vi "CSM-INI Variable Viewer - DebugTool.vi"(7 "Current Module(\"\" to generate an ID)":string="IniViewer") -> ()   [LabVIEW 2017]
doc: "CSM INI-Variable is a global configuration information. This tool is used to view and debug the current configuration information in memory.\n\n\n> [!NOTE] <b>CSM INI-Variable Addon</b>\n>\n> Configuration files are an essential component of application development. The CSM INI-Variable Addon provides simple and easy-to-use configuration file support for CSM, allowing users to configure applications without explicitly reading or writing configuration files.\n>\n> CSM INI-Variable configuration file data uses the CSM API String format.\n>\n> The following are key features:\n> 1. <b>Default Configuration Handling</b>: Automatically loads the default configuration file upon the first library function call, eliminating the need for explicit user loading.\n> 2. <b>Multi-File Support</b>: Supports loading multiple configuration files via specialized functions.\n> 3. <b>Memory Caching</b>: Maintains a cached copy in memory. Applications retrieve configuration information from this cache.\n> 4. <b>INI Format Compatibility</b>: Both configuration files and the memory copy use the standard INI format, supporting sections and key-value pairs.\n> 5. <b>Efficient Caching Mechanism</b>: Optimizes performance using a global modification flag, re-reading the memory copy only when the configuration has been modified.\n>\n> This library includes and utilizes a copy of [LabVIEW-Config](https://github.com/rcpacini/LabVIEW-Config) developed by [@rcpacini](https://github.com/rcpacini)."
uses:
  <userlib>/_NEVSTOP/Communicable State Machine(CSM)/_tool/_csmlite/_PassAllowedMessage - MsgList.vi
  _csm-iniViewer/csm-iniViewer.lvlib
  INI-Static-Variable-Support/INI-Static-Variable-Support.lvlib
  <userlib>/_NEVSTOP/Communicable State Machine(CSM)/_tool/_csmlite/_csmlite.lvlib
  <userlib>/_NEVSTOP/Communicable State Machine(CSM)/_tool/_ui/csm-ui-support.lvlib
panel:
  in  "Close":bool
  in  "Remove all Configurations":bool
  in  "Open":bool
  in  "Refresh":bool
  in  "Include Value?":bool
  in  "Filter":string
  in  "Tree":string(tree)
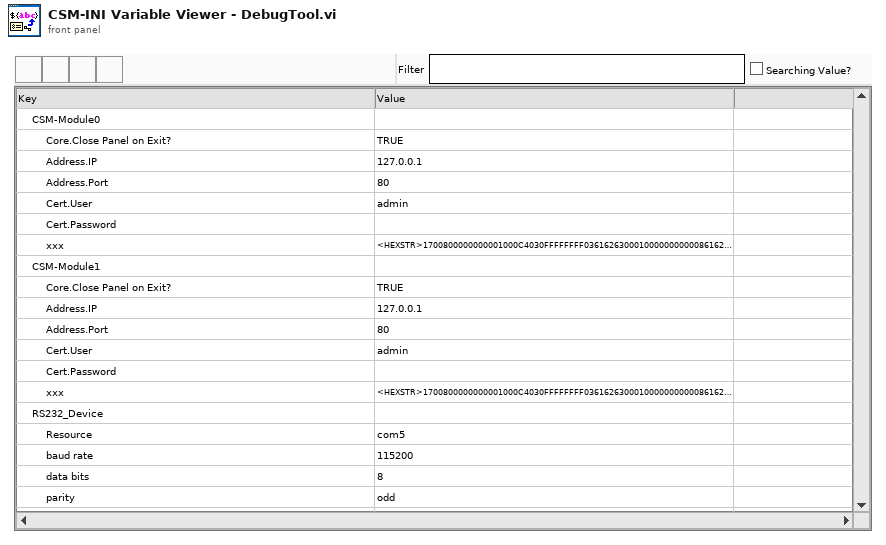
[diagram p1: front panel]
types:
  T1 = enum32{"Invalid", "Standard", "Closed", "Hidden", "Minimized", "Maximized"}
  T2 = enum32{"invalid app kind", "Development System", "Run Time System", "Student Edition", "Embedded LabVIEW", "Evaluation", "Custom"}
  T3 = cluster{"Core":cluster{"Current VI Reference":refnum<vi>, "Close Panel on Exit?":bool}, "Your Boolean data":bool, "Your string data":string}
  T4 = cluster{"Current VI Reference":refnum<vi>, "Close Panel on Exit?":bool}
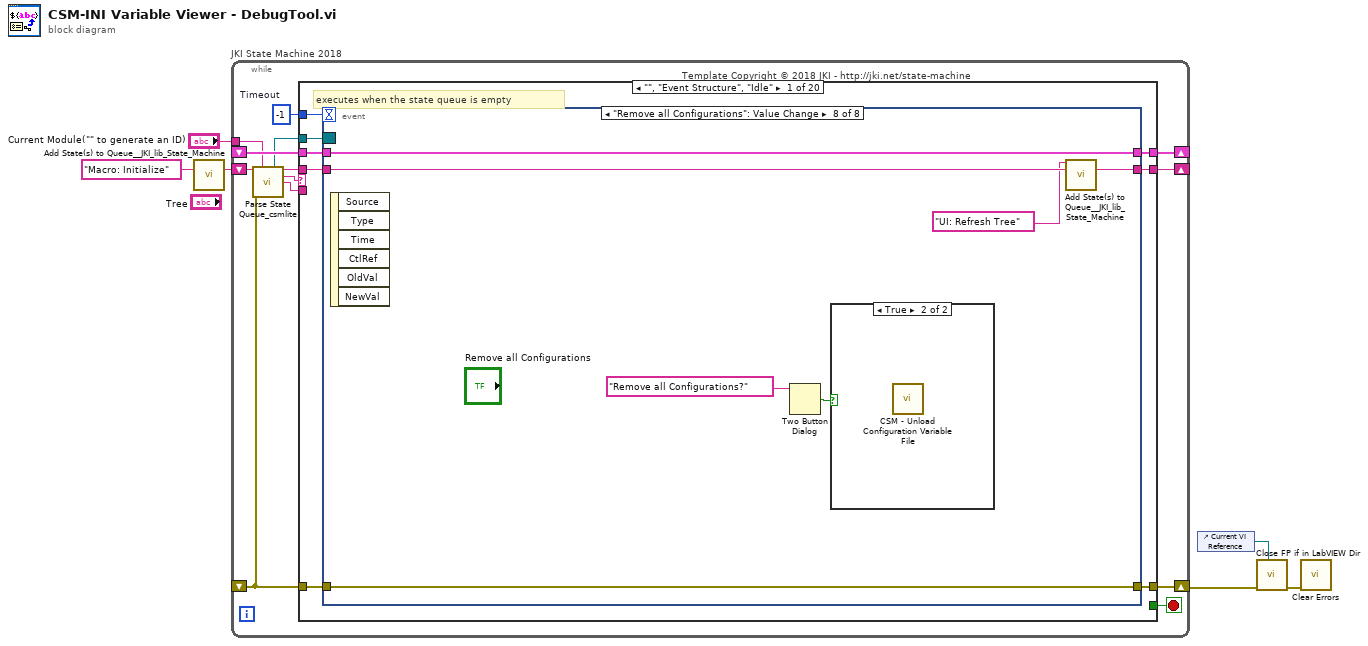
[diagram p0: block diagram]
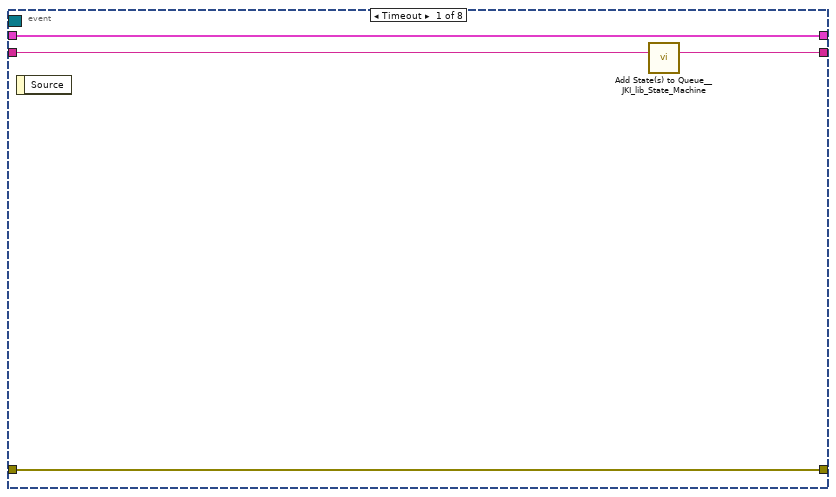
[diagram p2: hidden frame]
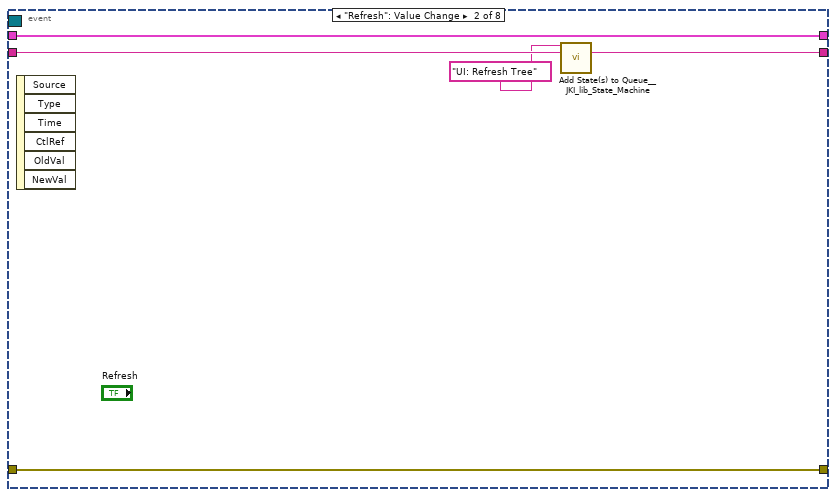
[diagram p3: hidden frame]
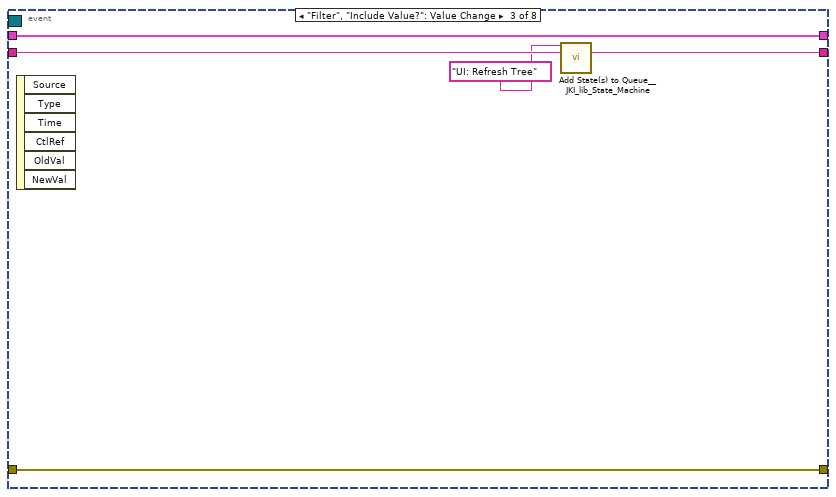
[diagram p4: hidden frame]
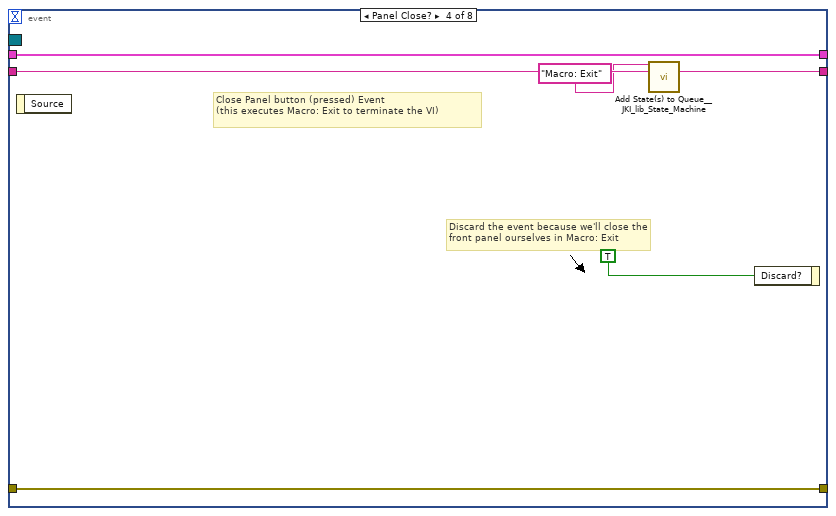
[diagram p5: hidden frame]
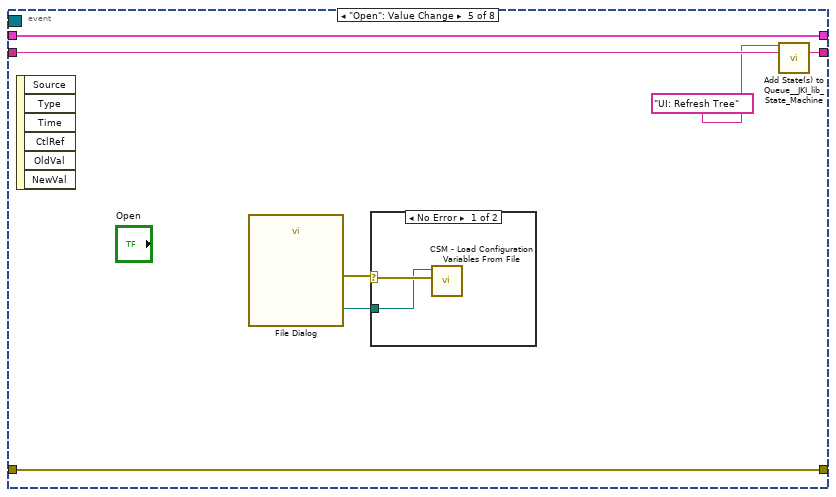
[diagram p6: hidden frame]
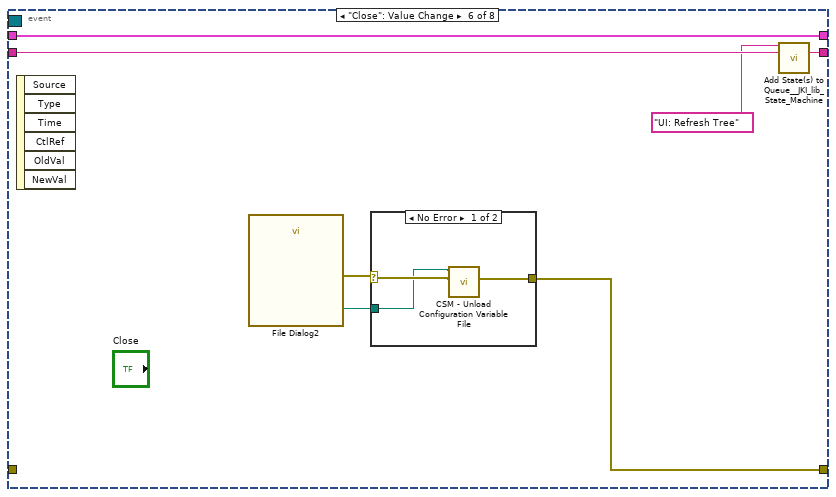
[diagram p8: hidden frame]
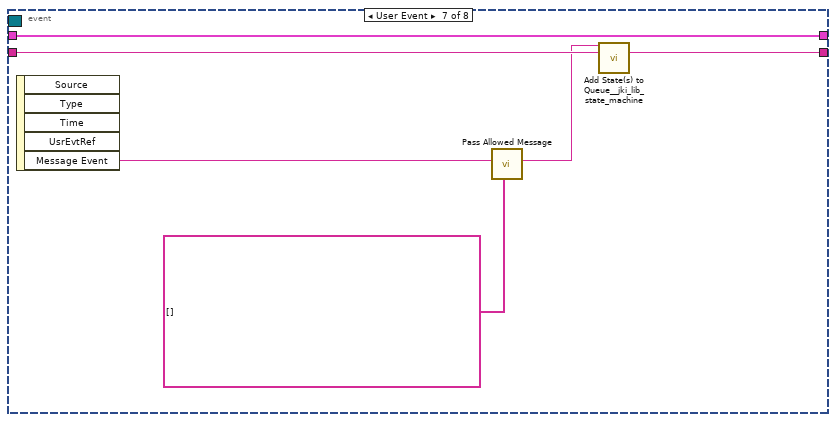
[diagram p10: hidden frame]
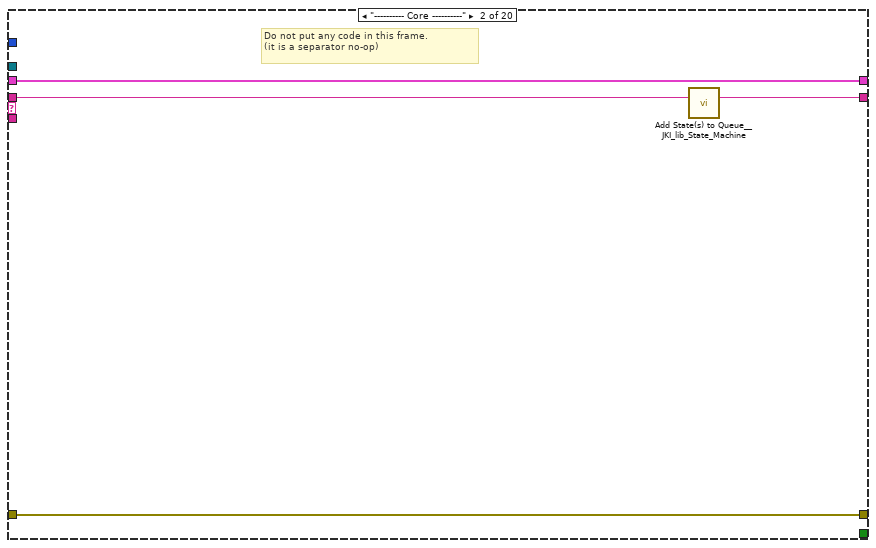
[diagram p12: hidden frame]
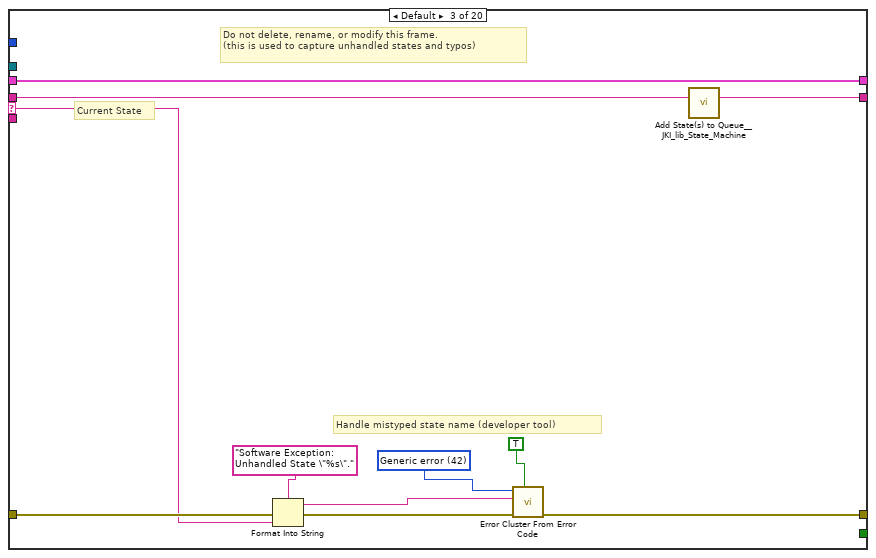
[diagram p13: hidden frame]
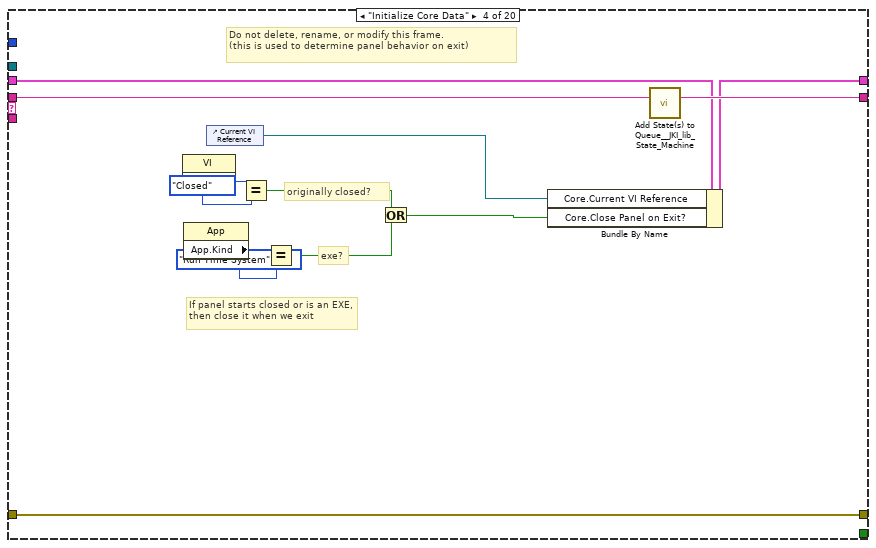
[diagram p14: hidden frame]
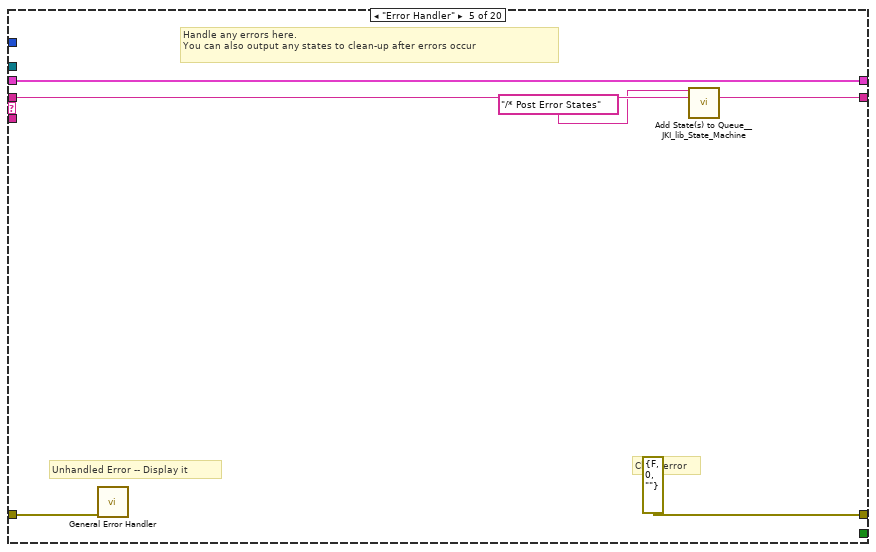
[diagram p15: hidden frame]
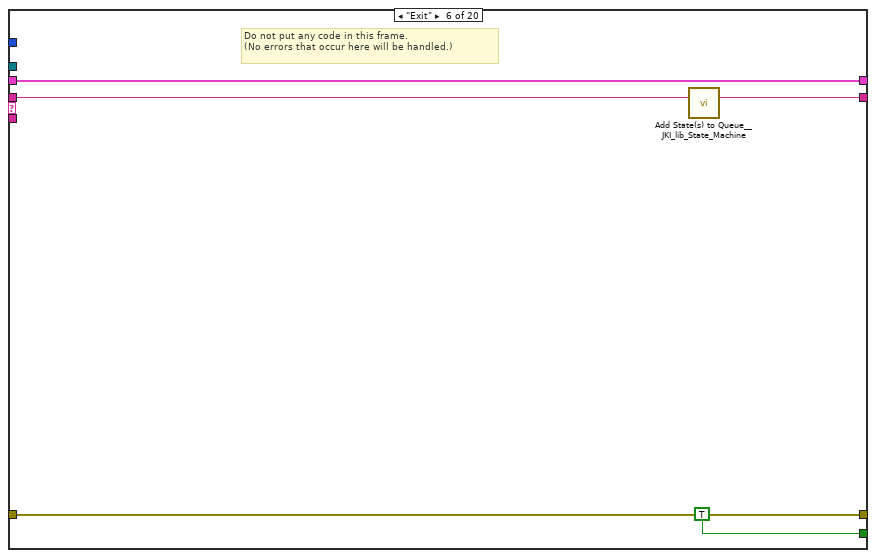
[diagram p16: hidden frame]
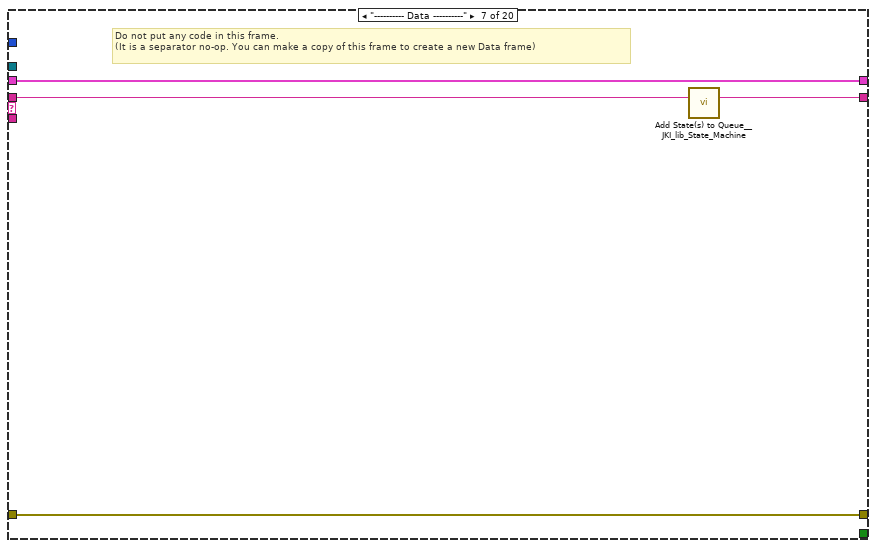
[diagram p17: hidden frame]
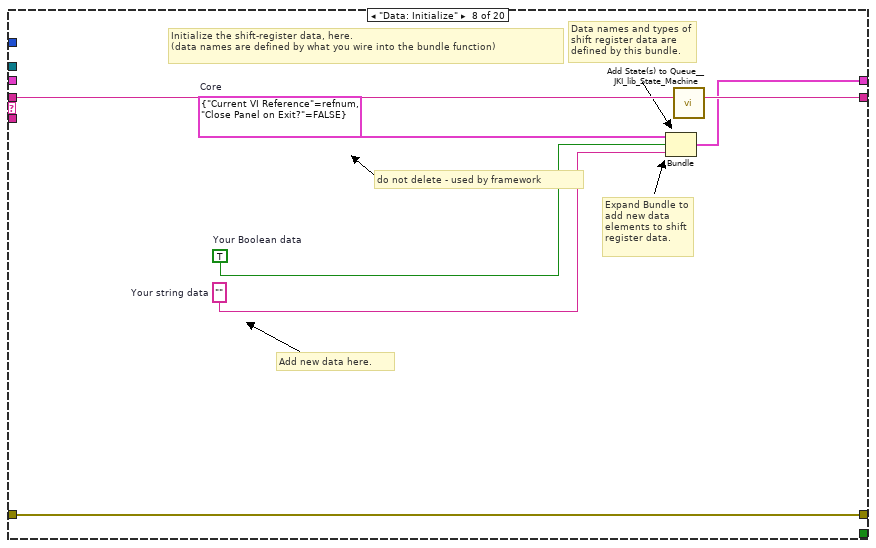
[diagram p18: hidden frame]
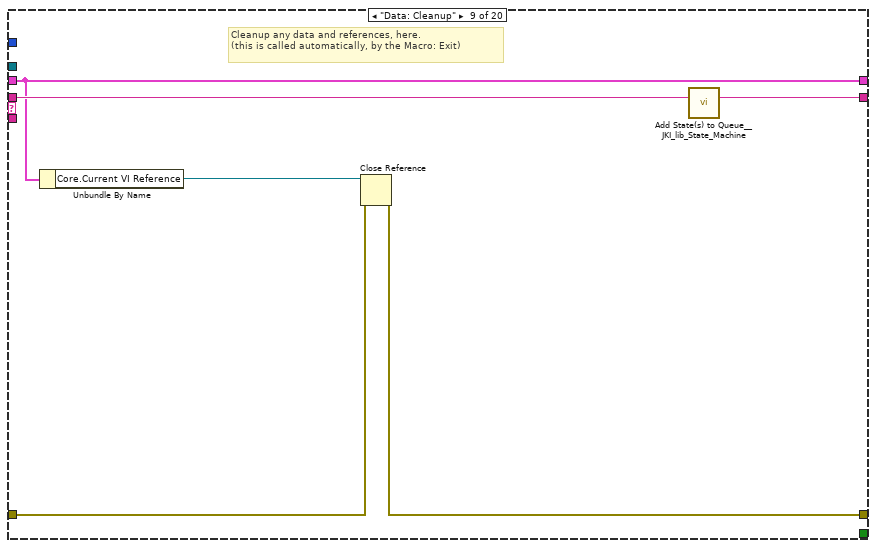
[diagram p19: hidden frame]
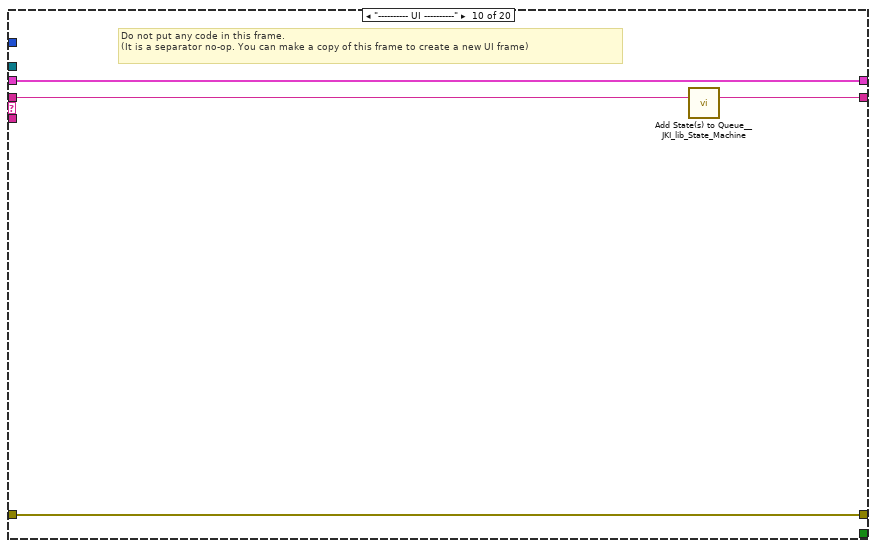
[diagram p20: hidden frame]
diagram:
  n1 = call <vilib>:"Add State(s) to Queue__JKI_lib_State_Machine.vi"("State(s) in (\"\")"="Macro: Initialize") -> ("States Out"=w6:string)  [unwired: 14 in]
  n2 = while "JKI State Machine 2018" {
    shift-right: [w12] -> _
    shift-left: _ -> [w11]
    shift-right: [w15] -> w3
    shift-left: _ -> [w9]
    shift-right: [w14] -> _
    shift-left: w6 -> [w16]
    tunnel: "Current Module(\"\" to generate an ID)" -> [w8]
    stop <- w13 stop-if-true
    w10 = -1  # Timeout
    # "Template Copyright © 2018 JKI - http://jki.net/state-machine"
    n3 = call <userlib>:"Parse State Queue_csmlite.vi"("State Queue"=w16, "Current Module(\"\" to generate an ID)"=w8, "Error In (no error)"=w9) -> ("Event Registration Refnum"=w7:refnum<event-registration>, "Remaining States"=w18:string, "Current State"=w19:string, "Arguments"=w17:string)  [unwired: 9 in]
    n4 = case shown="\"\", \"Event Structure\", \"Idle\"" w19 {
      selector: w19 -> [_ _ w84 _ _ _ _ _ _ _ _ _ _ _ _ _ _ _ _ _]
      tunnel: w18 -> [w27 w83 w88 w107 w113 w118 w122 w129 w135 w139 w151 w157 w168 w239 w243 w248 w258 w262 w266 w270]
      tunnel: w17 -> [_ _ _ _ _ _ _ _ _ _ _ w152 w162 _ _ _ _ _ _ _]
      tunnel: w11 -> [w25 w80 w86 w100 w110 w116 w119 _ w130 w136 w149 w155 w164 w238 w240 w245 w255 w259 w263 w267]
      tunnel: [w24 w81 w90 w104 errorcluster {"status"=FALSE, "code"=0, "source"=""} ("error out") w115 w120 w126 w131 w137 w148 w153 w165 w235 w241 w246 w256 w260 w264 w268] -> w15
      tunnel: w9 -> [w23 w81 w89 w104 w109 w115 w120 w126 w132 w137 w148 w154 w166 _ w241 w246 w256 w260 w264 w268]
      tunnel: [w26 w82 w87 w106 w112 w117 w121 w128 w134 w138 w150 w156 w167 w239 w242 w247 w257 w261 w265 w269] -> w14
      tunnel: [_ _ _ _ _ TRUE _ _ _ _ _ _ _ _ _ _ _ _ _ _] -> w13
      tunnel: [w22 w80 w86 w105 w110 w116 w119 w127 w130 w136 w149 w155 w164 w238 w240 w245 w255 w259 w263 w267] -> w12
      tunnel: w10 -> [w21 _ _ _ _ _ _ _ _ _ _ _ _ _ _ _ _ _ _ _]
      tunnel: w7 -> [w20 _ _ _ _ _ _ _ _ _ _ _ _ _ _ _ _ _ _ _]
      frame "", "Event Structure", "Idle" {
        # "executes when the state queue is empty"
        n5 = event shown="[7] \"Remove all Configurations\": Value Change" {
          selector: w20 -> [_ _ _ _ _ _ _ _]
          dyn-events: _ -> [_ _ _ _ _ _ _ _]
          timeout: w21 -> [_ _ _ _ _ _ _ _]
          tunnel: w27 -> [w31 w34 w39 w47 w49 w59 w68 w76]
          tunnel: [w30 w35 w40 w46 w50 w60 w69 w77] -> w26
          tunnel: w25 -> [w28 w36 w41 w44 w54 w63 w72 w79]
          tunnel: [w29 w32 w37 w45 w53 w57 _ w78] -> w24
          tunnel: w23 -> [w29 w32 w37 w45 w53 _ _ w78]
          tunnel: [w28 w36 w41 w44 w54 w63 w72 w79] -> w22
          event Timeout {
            n6 = event-data() -> ()  [unwired: 1 in, 1 out]
            n7 = call <vilib>:"Add State(s) to Queue__JKI_lib_State_Machine.vi"("State(s) in (\"\")"=w31) -> ("States Out"=w30:string)  [unwired: 14 in]
          }
          event "Refresh": Value Change {
            n8 = event-data() -> ()  [unwired: 1 in, 6 out]
            n9 = call <vilib>:"Add State(s) to Queue__JKI_lib_State_Machine.vi"("State(s) in Front (\"\")"="UI: Refresh Tree" ("State(s) in Front (\"\")"), "State(s) in (\"\")"=w34) -> ("States Out"=w35:string)  [unwired: 13 in]
          }
          event "Filter", "Include Value?": Value Change {
            n10 = event-data() -> ()  [unwired: 1 in, 6 out]
            n11 = call <vilib>:"Add State(s) to Queue__JKI_lib_State_Machine.vi"("State(s) in Front (\"\")"="UI: Refresh Tree" ("State(s) in Front (\"\")"), "State(s) in (\"\")"=w39) -> ("States Out"=w40:string)  [unwired: 13 in]
          }
          event Panel Close? {
            # "Discard the event because we'll close the front panel ourselves in Macro: Exit"
            # "Close Panel button (pressed) Event\n(this executes Macro: Exit to terminate the VI)"
            n12 = event-data() -> ()  [unwired: 1 in, 1 out]
            n13 = call <vilib>:"Add State(s) to Queue__JKI_lib_State_Machine.vi"("State(s) in Front (\"\")"="Macro: Exit", "State(s) in (\"\")"=w47) -> ("States Out"=w46:string)  [unwired: 13 in]
            n14 = event-data("Discard?"=TRUE) -> ()  [unwired: 1 in, 1 out]
          }
          event "Open": Value Change {
            n15 = event-data() -> ()  [unwired: 1 in, 6 out]
            n16 = call "File Dialog"() -> ("selected path"=w51:path, "error out"=w52:errorcluster)  [unwired: 12 in, 2 out]
            n17 = case shown="No Error" w52 {
              selector: w52 -> [w56 _]
              tunnel: w51 -> [w55 _]
              frame No Error {
                n18 = call "CSM - Load Configuration Variables From File.vi"("error in (no error)"=w56, "Configuration Path"=w55) -> ()  [unwired: 7 in, 1 out]
              }
              frame Error {
              }
            }
            n19 = call <vilib>:"Add State(s) to Queue__JKI_lib_State_Machine.vi"("State(s) in Front (\"\")"="UI: Refresh Tree" ("State(s) in Front (\"\")"), "State(s) in (\"\")"=w49) -> ("States Out"=w50:string)  [unwired: 13 in]
          }
          event "Close": Value Change {
            n20 = event-data() -> ()  [unwired: 1 in, 6 out]
            n21 = call "File Dialog2"() -> ("selected path"=w61:path, "error out"=w62:errorcluster)  [unwired: 12 in, 2 out]
            n22 = case shown="No Error" w62 {
              selector: w62 -> [w66 _]
              tunnel: w61 -> [w65 _]
              tunnel: [w64 _] -> w57
              frame No Error {
                n23 = call "CSM - Unload Configuration Variable File.vi"("error in (no error)"=w66, "Path"=w65) -> ("error out"=w64:errorcluster)  [unwired: 7 in]
              }
              frame Error {
              }
            }
            n24 = call <vilib>:"Add State(s) to Queue__JKI_lib_State_Machine.vi"("State(s) in Front (\"\")"="UI: Refresh Tree" ("State(s) in Front (\"\")"), "State(s) in (\"\")"=w59) -> ("States Out"=w60:string)  [unwired: 13 in]
          }
          event User Event {
            n25 = event-data() -> ("Message Event"=w70:string)  [unwired: 1 in, 4 out]
            n26 = call-poly <userlib>:"Pass Allowed Message.vi"("Allowed Message"=string[] [], "JKISM External Event"=w70) -> ("States"=w67:string)  [unwired: 7 in]
            n27 = call <vilib>:"Add State(s) to Queue__jki_lib_state_machine.vi"("State(s) in Front (\"\")"=w67, "State(s) in (\"\")"=w68) -> ("States Out"=w69:string)  [unwired: 13 in]
          }
          event "Remove all Configurations": Value Change {
            n28 = event-data() -> ()  [unwired: 1 in, 6 out]
            n29 = Two Button Dialog(message="Remove all Configurations?") -> (T button?=w74:bool)  [unwired: 2 in]
            n30 = case shown="True" w74 {
              frame False {
              }
              frame True {
                n31 = call "CSM - Unload Configuration Variable File.vi"() -> ()  [unwired: 9 in, 1 out]
              }
            }
            n32 = call <vilib>:"Add State(s) to Queue__JKI_lib_State_Machine.vi"("State(s) in Front (\"\")"="UI: Refresh Tree" ("State(s) in Front (\"\")"), "State(s) in (\"\")"=w76) -> ("States Out"=w77:string)  [unwired: 13 in]
          }
        }
      }
      frame "---------- Core ----------" {
        # "Do not put any code in this frame.\n(it is a separator no-op)"
        n33 = call <vilib>:"Add State(s) to Queue__JKI_lib_State_Machine.vi"("State(s) in (\"\")"=w83) -> ("States Out"=w82:string)  [unwired: 14 in]
      }
      frame Default {
        w93 = 42 items=["No error", "Argument error", "Memory is full", "Out of zone", "End of file", "File already open", "Generic file I/O error", "File not found", "File permission error", "Disk is full", "Duplicate path", "Too many files open", "System feature not enabled", "Resource file not found", "Cannot add resource", "Resource not found", "Image not found", "Image memory error", "Pen does not exist", "Config type invalid", "Config token not found", "Config parse error", "Config memory error", "Bad external code format", "Bad external code offset", "External code not present", "Null window", "Destroy window error", "Null menu", "Print aborted", "Bad print record", "Print driver error", "Windows error during printing", "Memory error during printing", "Print dialog error", "Generic print error", "Invalid device refnum", "Device not found", "Device parameter error", "Device unit error", "Cannot open device", "Device call aborted", "Generic error", "Cancelled by user", "Object ID too low", "Object ID too high", "Object not in heap", "Unknown heap", "Unknown object (invalid DefProc)", "Unknown object (DefProc not in table)", "Message out of range", "Invalid (null) method", "Unknown message", "Manager call not supported", "Bad address", "Network operation in progress", "Network operation timed out", "Connection is busy", "Network attribute not supported", "Network error", "Address in use", "System out of memory", "Connection aborted", "Connection refused", "Not connected", "Already connected", "Connection closed", "Initialization error (interapplication manager)", "Bad occurrence", "Wait on unbound occurrence handler", "Occurrence queue overflow", "Datalog type conflict", "Unused", "Unrecognized type (interapplication manager)", "Memory corrupt", "Failed to make temporary DLL", "Old CIN version", "Drag socket not found", "Failed to load drop-object", "Failed to register OLE object", "Failed to release OLE object", "Format specifier type mismatch", "Unknown format specifier", "Too few format specifiers", "Too many format specifiers", "Scan failed", "Newer CIN version", "Error converting to variant", "Runtime menu error", "Password tampered", "Variant attribute not found", "Incompatible variant data type", "Event data is not available", "Event Store is not present", "Occurrence is not found", "Event Queue is not created", "Event info is not available", "Refnum passed is NULL", "Error retrieving Class GUID", "Error retrieving CoClass GUID", "Error retrieving TypeLib GUID.", "Bad built application magic bytes.", "Specific driver is different from the specific driver associated with the Logical Name.", "There is no session opened to the class driver.", "Max Error", "MAX - Error with config objects", "MAX - Error loading configuration", "MAX - Group not supported"]
        # "Current State"
        # "Do not delete, rename, or modify this frame.\n(this is used to capture unhandled states and typos)"
        # "Handle mistyped state name (developer tool)"
        n34 = Format Into String(format string="Software Exception: Unhandled State \"%s\"." ("message"), error in=w89, w84) -> (resulting string=w92:string, error out=w91:errorcluster)  [unwired: 1 in]
        n35 = call <vilib>:"Error Cluster From Error Code.vi"("show call chain? (False)"=TRUE, "error in (no error)"=w91, "error message (\"\")"=w92, "error code (0)"=w93) -> ("error out"=w90:errorcluster)  [unwired: 5 in]
        n36 = call <vilib>:"Add State(s) to Queue__JKI_lib_State_Machine.vi"("State(s) in (\"\")"=w88) -> ("States Out"=w87:string)  [unwired: 14 in]
      }
      frame "Initialize Core Data" {
        # "Do not delete, rename, or modify this frame.\n(this is used to determine panel behavior on exit)"
        # "originally closed?"
        # "exe?"
        # "If panel starts closed or is an EXE, then close it when we exit"
        n37 = property class="VI"() -> ("FP.State"=w97:T1)  [unwired: 2 in, 2 out]
        n38 = property class="App"() -> ("App.Kind"=w103:T2)  [unwired: 2 in, 2 out]
        n39 = control-ref of="Current VI Reference"() -> (w98:refnum<vi>)
        n40 = Equal?(x=w97, y=T1."Closed" ("Front Panel Window:State")) -> (x = y?=w95:bool)
        n41 = Equal?(x=w103, y=T2."Run Time System" ("Application:Kind")) -> (x = y?=w101:bool)
        n42 = Or(x=w95, y=w101) -> (x .or. y?=w99:bool)
        n43 = Bundle By Name(cluster=w100, "Core.Current VI Reference"=w98, "Core.Close Panel on Exit?"=w99) -> (w105:T3)
        n44 = call <vilib>:"Add State(s) to Queue__JKI_lib_State_Machine.vi"("State(s) in (\"\")"=w107) -> ("States Out"=w106:string)  [unwired: 14 in]
      }
      frame "Error Handler" {
        # "Unhandled Error -- Display it"
        # "Handle any errors here.\nYou can also output any states to clean-up after errors occur"
        # "Clear error"
        n45 = call <vilib>:"General Error Handler.vi"("error in (no error)"=w109) -> ()  [unwired: 10 in, 5 out]
        n46 = call <vilib>:"Add State(s) to Queue__JKI_lib_State_Machine.vi"("State(s) in Front (\"\")"="/* Post Error States", "State(s) in (\"\")"=w113) -> ("States Out"=w112:string)  [unwired: 13 in]
      }
      frame "Exit" {
        # "Do not put any code in this frame.\n(No errors that occur here will be handled.)"
        n47 = call <vilib>:"Add State(s) to Queue__JKI_lib_State_Machine.vi"("State(s) in (\"\")"=w118) -> ("States Out"=w117:string)  [unwired: 14 in]
      }
      frame "---------- Data ----------" {
        # "Do not put any code in this frame.\n(It is a separator no-op. You can make a copy of this frame to create a new Data frame)"
        n48 = call <vilib>:"Add State(s) to Queue__JKI_lib_State_Machine.vi"("State(s) in (\"\")"=w122) -> ("States Out"=w121:string)  [unwired: 14 in]
      }
      frame "Data: Initialize" {
        w123 = T4 {"Current VI Reference"=refnum, "Close Panel on Exit?"=FALSE}  # Core
        w125 = TRUE  # Your Boolean data
        w124 = ""  # Your string data
        # "do not delete - used by framework"
        # "Expand Bundle to add new data elements to shift register data."
        # "Add new data here."
        # "Data names and types of shift register data are defined by this bundle."
        # "Initialize the shift-register data, here.\n(data names are defined by what you wire into the bundle function)"
        n49 = Bundle("Core"=w123, "Your Boolean data"=w125, "Your string data"=w124) -> (w127:T3)  [unwired: 1 in]
        n50 = call <vilib>:"Add State(s) to Queue__JKI_lib_State_Machine.vi"("State(s) in (\"\")"=w129) -> ("States Out"=w128:string)  [unwired: 14 in]
      }
      frame "Data: Cleanup" {
        # "Cleanup any data and references, here.\n(this is called automatically, by the Macro: Exit)"
        n51 = Unbundle By Name(w130) -> ("Core.Current VI Reference"=w133:refnum<vi>)
        n52 = Close Reference(reference=w133, error in (no error)=w132) -> (error out=w131:errorcluster)
        n53 = call <vilib>:"Add State(s) to Queue__JKI_lib_State_Machine.vi"("State(s) in (\"\")"=w135) -> ("States Out"=w134:string)  [unwired: 14 in]
      }
      frame "---------- UI ----------" {
        # "Do not put any code in this frame.\n(It is a separator no-op. You can make a copy of this frame to create a new UI frame)"
        n54 = call <vilib>:"Add State(s) to Queue__JKI_lib_State_Machine.vi"("State(s) in (\"\")"=w139) -> ("States Out"=w138:string)  [unwired: 14 in]
      }
      frame "UI: Initialize" {
        # "Initialize the User Interface, here.\n(this is called automatically, by the Macro: Init)"
        n55 = call "CSM - Configuration File Path.vi"() -> ("Default Config File Path"=w143:path)  [unwired: 7 in, 2 out]
        n56 = control-ref of="Tree"() -> (w147:refnum<vi>)
        n57 = Path To String(path=w143) -> (string=w142:string)
        n58 = Concatenate Strings("Default Configuration Path: " ("string"), w142) -> (w141:string)
        n59 = invoke on="Invoke Node" class="Tree (strict)" method="Edit Tree Items.Delete"(reference=w147, "tag"="" ("Tag"), "Delete Children"=TRUE ("Delete Children?")) -> ()  [unwired: 2 in, 5 out]
        n60 = local write "Filter"("" ("Filter")) -> ()
        n61 = property class="VI"("Front Panel.Title"=w141) -> ()  [unwired: 2 in, 2 out]
        n62 = call <vilib>:"Add State(s) to Queue__JKI_lib_State_Machine.vi"("State(s) in (\"\")"=w151) -> ("States Out"=w150:string)  [unwired: 14 in]
      }
      frame "UI: Cursor Set" {
        # "Argument"
        # "Set and Unset Cursor Busy.\n(Usage: \"UI: Cursor Set >> Busy|Idle\")"
        n63 = case shown="\"Idle\", Default" w152 {
          tunnel: w154 -> [w159 w161]
          tunnel: [w158 w160] -> w153
          frame "Idle", Default {
            n64 = call <vilib>:"Unset Busy.vi"("error in (no error)"=w159) -> ("error out"=w158:errorcluster)  [unwired: 10 in]
          }
          frame "Busy" {
            n65 = call <vilib>:"Set Busy.vi"("error in (no error)"=w161) -> ("error out"=w160:errorcluster)  [unwired: 9 in, 1 out]
          }
        }
        n66 = call <vilib>:"Add State(s) to Queue__JKI_lib_State_Machine.vi"("State(s) in (\"\")"=w157) -> ("States Out"=w156:string)  [unwired: 14 in]
      }
      frame "UI: Front Panel State" {
        # "Argument"
        # "Set Front Panel Open or Closed\n(Usage: \"UI: Front Panel State >> Open|Close\")"
        n67 = Unbundle By Name(w164) -> ("Core.Current VI Reference"=w163:refnum<vi>)
        n68 = case shown="\"Minimize\", \"Minimized\"" w162 {
          tunnel: w166 -> [w174 w189 w200 w213 w226]
          tunnel: [w176 w190 w202 w215 w228] -> w165
          tunnel: w163 -> [w175 w187 w201 w214 w227]
          frame "Open", "Standard", Default {
            w169 = T1."Standard" ("State")
            n69 = property class="VI"(reference=w175, error in=w174) -> (reference out=w172:refnum<vi>, error out=w173:errorcluster, "FP.State"=w171:T1)
            n70 = Not Equal?(x=w171, y=w169) -> (x != y?=w170:bool)
            n71 = case shown="True" w170 {
              tunnel: [w180 w182] -> w176
              tunnel: w173 -> [w179 w182]
              tunnel: w172 -> [w178 _]
              tunnel: w169 -> [w177 _]
              frame True {
                n72 = invoke class="VI" method="FP.Open"(reference=w178, error in=w179, "Activate"=TRUE, "State"=w177) -> (error out=w180:errorcluster)  [unwired: 1 in, 4 out]
              }
              frame False {
              }
            }
          }
          frame "Close", "Closed" {
            n73 = property class="VI"(reference=w187, error in=w189) -> (reference out=w186:refnum<vi>, error out=w188:errorcluster, "FP.State"=w184:T1)
            n74 = Not Equal?(x=w184, y=T1."Closed" ("Front Panel Window:State")) -> (x != y?=w183:bool)
            n75 = case shown="True" w183 {
              tunnel: [w191 w194] -> w190
              tunnel: w188 -> [w191 w193]
              tunnel: w186 -> [_ w192]
              frame False {
              }
              frame True {
                n76 = invoke class="VI" method="FP.Close"(reference=w192, error in=w193) -> (error out=w194:errorcluster)  [unwired: 1 in, 2 out]
              }
            }
          }
          frame "Hidden", "Hide" {
            w195 = T1."Hidden" ("State")
            n77 = property class="VI"(reference=w201, error in=w200) -> (reference out=w198:refnum<vi>, error out=w199:errorcluster, "FP.State"=w197:T1)
            n78 = Not Equal?(x=w197, y=w195) -> (x != y?=w196:bool)
            n79 = case shown="True" w196 {
              tunnel: [w206 w207] -> w202
              tunnel: w199 -> [w205 w207]
              tunnel: w198 -> [w204 _]
              tunnel: w195 -> [w203 _]
              frame True {
                n80 = invoke class="VI" method="FP.Open"(reference=w204, error in=w205, "State"=w203) -> (error out=w206:errorcluster)  [unwired: 2 in, 4 out]
              }
              frame False {
              }
            }
          }
          frame "Minimize", "Minimized" {
            w208 = T1."Minimized" ("State")
            n81 = property class="VI"(reference=w214, error in=w213) -> (reference out=w211:refnum<vi>, error out=w212:errorcluster, "FP.State"=w210:T1)
            n82 = Not Equal?(x=w210, y=w208) -> (x != y?=w209:bool)
            n83 = case shown="True" w209 {
              tunnel: [w219 w220] -> w215
              tunnel: w212 -> [w218 w220]
              tunnel: w211 -> [w217 _]
              tunnel: w208 -> [w216 _]
              frame True {
                n84 = invoke class="VI" method="FP.Open"(reference=w217, error in=w218, "State"=w216) -> (error out=w219:errorcluster)  [unwired: 2 in, 4 out]
              }
              frame False {
              }
            }
          }
          frame "Maximize", "Maximized" {
            w221 = T1."Maximized" ("State")
            n85 = property class="VI"(reference=w227, error in=w226) -> (reference out=w224:refnum<vi>, error out=w225:errorcluster, "FP.State"=w223:T1)
            n86 = Not Equal?(x=w223, y=w221) -> (x != y?=w222:bool)
            n87 = case shown="True" w222 {
              tunnel: [w232 w233] -> w228
              tunnel: w225 -> [w231 w233]
              tunnel: w224 -> [w230 _]
              tunnel: w221 -> [w229 _]
              frame True {
                n88 = invoke class="VI" method="FP.Open"(reference=w230, error in=w231, "State"=w229) -> (error out=w232:errorcluster)  [unwired: 2 in, 4 out]
              }
              frame False {
              }
            }
          }
        }
        n89 = call <vilib>:"Add State(s) to Queue__JKI_lib_State_Machine.vi"("State(s) in (\"\")"=w168) -> ("States Out"=w167:string)  [unwired: 14 in]
      }
      frame "UI: Refresh Tree" {
        n90 = control-ref of="Tree"() -> (w236:refnum<vi>)
        n91 = call "Populate all INI Variables to Tree.vi"("Include Value?"="Include Value?", "Filter"="Filter", "TreeControl in"=w236) -> ("Error out"=w235:errorcluster)  [unwired: 8 in]
      }
      frame "---------- Macro ----------" {
        # "Do not put any code in this frame.\n(It is a separator no-op. You can make a copy of this frame to create a new Macro frame)"
        n92 = call <vilib>:"Add State(s) to Queue__JKI_lib_State_Machine.vi"("State(s) in (\"\")"=w243) -> ("States Out"=w242:string)  [unwired: 14 in]
      }
      frame "Macro: Initialize" {
        w244 = "Data: Initialize\nInitialize Core Data\nUI: Initialize\n//UI: Front Panel State >> Open\nUI: Refresh Tree"  # Data: Initialize Initialize Core Data UI: Initialize //UI: Front Panel State >> Open UI: Refresh Tree
        # "Initialization Macro\n(This is called once, when the VI starts)"
        n93 = call <vilib>:"Add State(s) to Queue__JKI_lib_State_Machine.vi"("State(s) in Front (\"\")"=w244, "State(s) in (\"\")"=w248) -> ("States Out"=w247:string)  [unwired: 13 in]
      }
      frame "Macro: Exit" {
        # "Exit Macro\n(This is called once, when the VI exits)"
        n94 = Unbundle By Name(w255) -> ("Core.Close Panel on Exit?"=w254:bool)
        n95 = Select(t="UI: Front Panel State >> Close", s=w254, f="") -> (s? t:f=w251:string)
        n96 = call <vilib>:"Add State(s) to Queue__JKI_lib_State_Machine.vi"("State(s) in (\"\")"=w251, "State(s) at Back (\"\")"="Data: Cleanup\nExit") -> ("States Out"=w249:string)  [unwired: 13 in]
        n97 = call <vilib>:"Add State(s) to Queue__JKI_lib_State_Machine.vi"("State(s) in Front (\"\")"=w249, "State(s) in (\"\")"=w258) -> ("States Out"=w257:string)  [unwired: 13 in]
      }
      frame "---------- New Category ----------" {
        # "Template Separator\n(You can make a copy of, or modify, this frame)"
        n98 = call <vilib>:"Add State(s) to Queue__JKI_lib_State_Machine.vi"("State(s) in (\"\")"=w262) -> ("States Out"=w261:string)  [unwired: 14 in]
      }
      frame "New Category: 1" {
        # "Your code here.\n(You can make a copy of, or modify, this frame)"
        n99 = call <vilib>:"Add State(s) to Queue__JKI_lib_State_Machine.vi"("State(s) in (\"\")"=w266) -> ("States Out"=w265:string)  [unwired: 14 in]
      }
      frame "New Category: 2" {
        # "Your code here.\n(You can make a copy of, or modify, this frame)"
        n100 = call <vilib>:"Add State(s) to Queue__JKI_lib_State_Machine.vi"("State(s) in (\"\")"=w270) -> ("States Out"=w269:string)  [unwired: 14 in]
      }
    }
  }
  n101 = control-ref of="Current VI Reference"() -> (w2:refnum<vi>)
  n102 = call <userlib>:"Close FP if in LabVIEW Dir.vi"("VI Refnum"=w2, "Error in"=w3) -> ("Error out"=w1:errorcluster)  [unwired: 9 in]
  n103 = call <vilib>:"Clear Errors.vi"("error in (no error)"=w1) -> ()  [unwired: 5 in, 2 out]
